vi "Plugin_Poll.vi"(8 "error in (no error)":errorcluster={"status"=FALSE, "code"=0, "source"="\"\""}, 10 "latest status":string, 11 "Instance ID":string) -> (0 "error out":errorcluster={"status"=FALSE, "code"=0, "source"="\"\""}, 2 "status ok":bool, 3 "Active/completed/unresponsive":string)   [LabVIEW 2026]
doc: "INTENT: Monitor worker responsiveness. LOGIC: Check heartbeat and bounded progress updates; report missed deadlines to Supervisor."
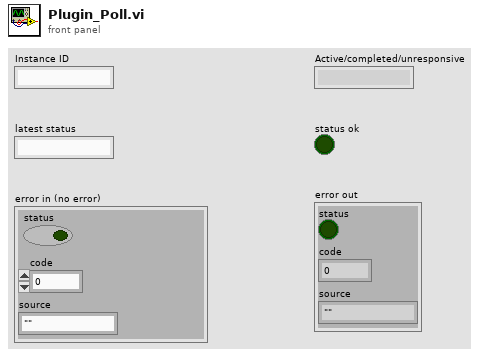
[diagram p1: front panel]
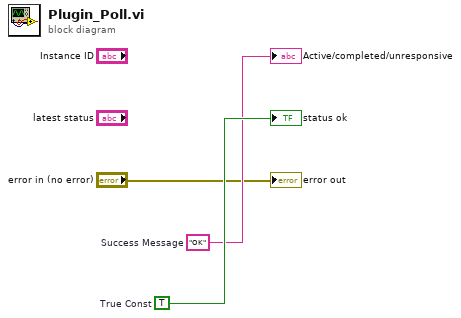
[diagram p0: block diagram]
diagram:
  w3 = TRUE  # True Const
  w2 = "OK"  # Success Message
  "Active/completed/unresponsive" <- w2
  "status ok" <- w3
  "error out" <- "error in (no error)"
